vi "Roll_Dice.vi"() -> ()   [LabVIEW 2026]
uses:
  SubVIs/Dice_face.ctl
panel:
  out "6":string
  out "5":string
  out "4":string
  out "3":string
  out "2":string
  out "Face:":string
  out "Roll Count":i32[](array[numeric]) caption="Roll Count's"
  out "Last 10 Roll's":i32[](array[numeric])
  out "Total Roll Count":dbl
  out "Roll Results":dbl[](graph)
  out "?":T1
  out "ESP32 Connected":bool
  out "Roll Result":i32
  in  "ESP32 Comm Port:":refnum<visa-resource-name>
  in  "STOP":bool
  in  "Roll (1-6)":bool
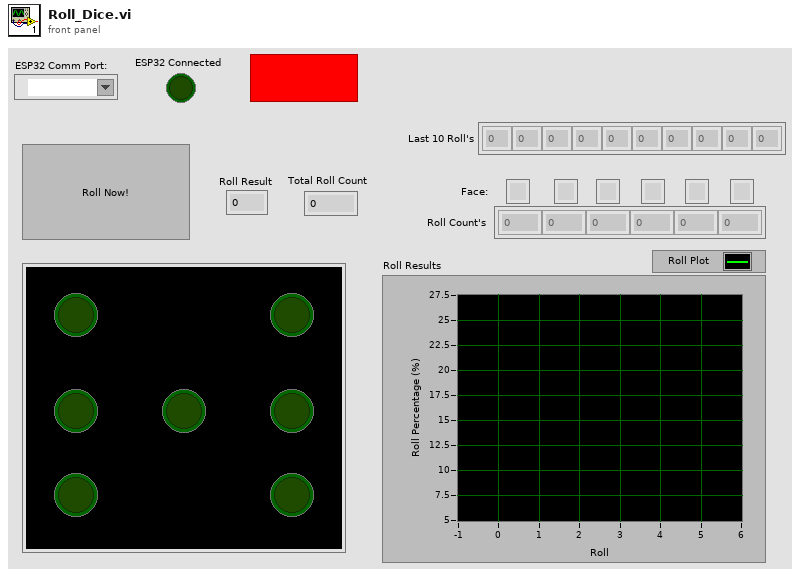
[diagram p1: front panel]
types:
  T1 = typedef "Dice_face.ctl" = cluster{"Boolean":bool, "Boolean 5":bool, "Boolean 6":bool, "Boolean 2":bool, "Boolean 3":bool, "Boolean 4":bool, "Boolean 7":bool}
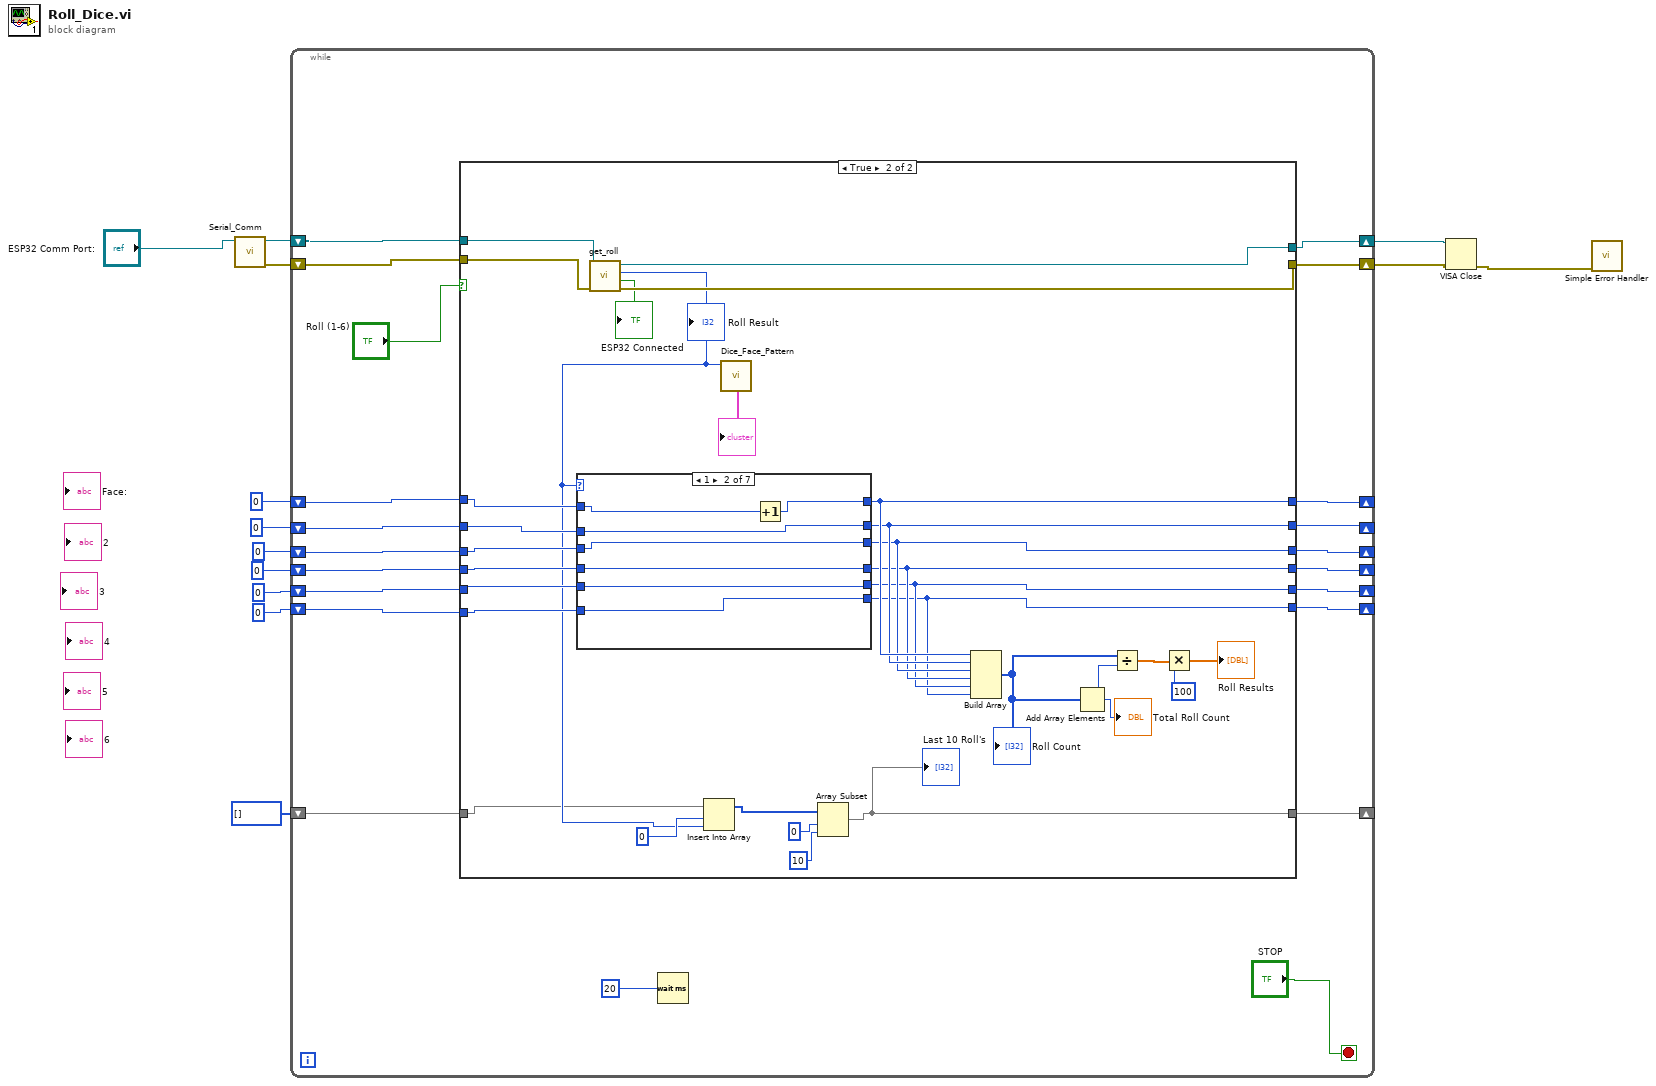
[diagram p0: block diagram]
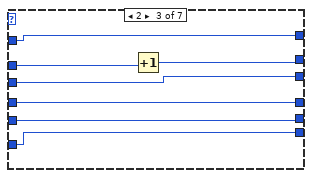
[diagram p4: hidden frame]
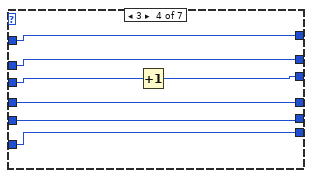
[diagram p5: hidden frame]
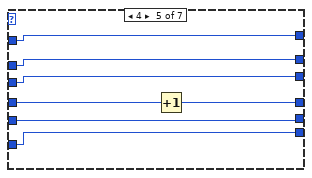
[diagram p6: hidden frame]
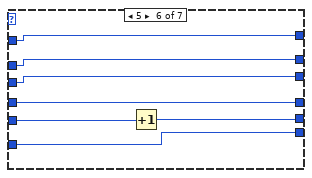
[diagram p7: hidden frame]
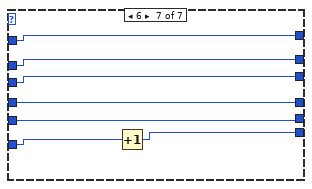
[diagram p8: hidden frame]
diagram:
  n1 = call "Serial_Comm.vi"("ESP32_Data"="ESP32 Comm Port:") -> ("Roll_result"=w12:refnum<visa-resource-name>, "error out"=w11:errorcluster)  [unwired: 8 in]
  n2 = while {
    shift-right: [w31] -> w10
    shift-left: w12 -> [w34]
    shift-right: [w30] -> w9
    shift-left: w11 -> [w33]
    shift-right: [w21] -> _
    shift-left: 0 -> [w27]
    shift-right: [w20] -> _
    shift-left: 0 -> [w26]
    shift-right: [w19] -> _
    shift-left: 0 -> [w25]
    shift-right: [w18] -> _
    shift-left: 0 -> [w24]
    shift-right: [w17] -> _
    shift-left: 0 -> [w23]
    shift-right: [w16] -> _
    shift-left: 0 -> [w22]
    shift-right: [w14] -> _
    shift-left: i32[] [] -> [w15]
    stop <- "STOP" stop-if-true
    n3 = case shown="True" "Roll (1-6)" {
      tunnel: w34 -> [w43 w73]
      tunnel: w33 -> [w42 w72]
      tunnel: [w43 w68] -> w31
      tunnel: [w42 w71] -> w30
      tunnel: w27 -> [w41 w67]
      tunnel: w26 -> [w40 w66]
      tunnel: w25 -> [w39 w65]
      tunnel: w24 -> [w38 w64]
      tunnel: w23 -> [w37 w63]
      tunnel: w22 -> [w36 w62]
      tunnel: [w41 w59] -> w21
      tunnel: [w40 w58] -> w20
      tunnel: [w39 w57] -> w19
      tunnel: [w38 w56] -> w18
      tunnel: [w37 w55] -> w17
      tunnel: [w36 w54] -> w16
      tunnel: w15 -> [w35 w45]
      tunnel: [w35 w44] -> w14
      frame False {
      }
      frame True {
        n4 = call "get_roll.vi"("error in (no error)"=w72, "ESP32 TRNG"=w73) -> ("error out"=w71:errorcluster, "from ESP32?"=→"ESP32 Connected":bool, "roll"=w49:i32, "ESP32 TRNG"=w68:refnum<visa-resource-name>)  [unwired: 6 in]
        "Roll Result" <- w49
        n5 = case shown="1" w49 {
          tunnel: [w79 w85 w93 w100 w105 w108 w115] -> w59
          tunnel: w67 -> [w79 w86 w93 w100 w105 w108 w115]
          tunnel: w66 -> [w78 w84 w92 w99 w104 w109 w116]
          tunnel: [w78 w84 w91 w99 w104 w109 w116] -> w58
          tunnel: w65 -> [w77 w83 w90 w98 w103 w110 w117]
          tunnel: [w77 w83 w90 w97 w103 w110 w117] -> w57
          tunnel: [w76 w82 w89 w96 w106 w111 w118] -> w56
          tunnel: w64 -> [w76 w82 w89 w96 w107 w111 w118]
          tunnel: [w75 w81 w88 w95 w102 w113 w119] -> w55
          tunnel: w63 -> [w75 w81 w88 w95 w102 w114 w119]
          tunnel: w62 -> [w74 w80 w87 w94 w101 w112 w121]
          tunnel: [w74 w80 w87 w94 w101 w112 w120] -> w54
          frame 0, Default {
          }
          frame 1 {
            n6 = Increment(x=w86) -> (x+1=w85:i32)
          }
          frame 2 {
            n7 = Increment(x=w92) -> (x+1=w91:i32)
          }
          frame 3 {
            n8 = Increment(x=w98) -> (x+1=w97:i32)
          }
          frame 4 {
            n9 = Increment(x=w107) -> (x+1=w106:i32)
          }
          frame 5 {
            n10 = Increment(x=w114) -> (x+1=w113:i32)
          }
          frame 6 {
            n11 = Increment(x=w121) -> (x+1=w120:i32)
          }
        }
        n12 = Insert Into Array(array=w45, index=0, new element=w49) -> (w48:i32[])
        n13 = call "Dice_Face_Pattern.vi"("Numeric"=w49) -> ("Cluster"=→"?":T1)  [unwired: 10 in]
        n14 = Array Subset(array=w48, index=0, length=10) -> (w44:i32[])
        "Last 10 Roll's" <- w44
        n15 = Build Array(w59, w58, w57, w56, w55, w54) -> (w52:i32[])
        "Roll Count" <- w52
        n16 = Add Array Elements(numeric array=w52) -> (sum=w51:i32)
        "Total Roll Count" <- w51
        n17 = Divide(x=w52, y=w51) -> (x/y=w60:dbl[])
        n18 = Multiply(x=w60, y=100) -> (x*y=→"Roll Results":dbl[])
      }
    }
    n19 = Wait (ms)(milliseconds to wait=u32 20) -> ()  [unwired: 1 out]
  }
  n20 = VISA Close(VISA resource name=w10, error in (no error)=w9) -> (error out=w8:errorcluster)
  n21 = call <vilib>:"Simple Error Handler.vi"("error in (no error)"=w8) -> ()  [unwired: 4 in, 5 out]
